vi "Set Translation.vi"(8 "error in (no error)":errorcluster, 9 "Default Lang":i32, 10 "Language":T1) -> (0 "error out":errorcluster)   [LabVIEW 2019, in "Language Selection.lvlib"]
doc: "Sets the translation of the VI controls according to the \"Language\" input index.\n- - -\nCopyright (c) 2026, Merecs Engineering GmbH"
uses:
  Language Selection.lvlib
  TypeDefs/Enum Language.ctl
  <vilib>/Utility/error.llb/Clear Errors.vi
  Set use unicode and default Lang.vi
  <vilib>/Utility/error.llb/Trim Whitespace.vi
  DVR Get Languages.vi
  Boolean Translate.vi
  Update Controls/Update MC Listbox vColumn headers.vi
  Update Controls/Update Listbox headers.vi
  Update Controls/Tool_Unicode Update Table Headers.vi
  Update Controls/update Graph.vi
  Update Controls/update 1D array.vi
  Update Controls/update tree column header.vi
  Update Controls/update 2D array.vi
  Update Controls/update listbox Items.vi
  Update Controls/update MultiColumn Listbox Items.vi
  Update Controls/Tool_Unicode Update Table Data.vi
  Update Controls/Update caption.vi
  Update Controls/update ring.vi
  <vilib>/addons/Tools/Unicode/Property Interpret As Unicode.vi
  <vilib>/addons/Tools/Unicode/Convert ASCII to UTF-16LE.vi
  <vilib>/addons/Tools/Unicode/_subVIs/Convert ASCII to UTF-16LE (1D).vi
  Update Controls/Update String value.vi
  Update Controls/Tool_Unicode Update Tab Control Pages.vi
  packages/error-generation/src/Error Generation/Add Argument.vi
panel:
  # "Connector Pane"
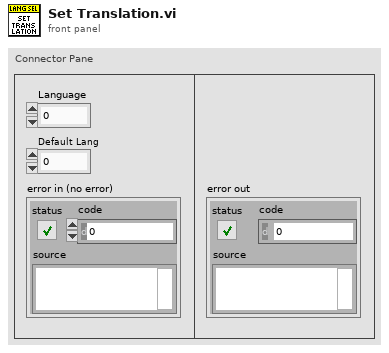
[diagram p1: front panel]
types:
  T1 = typedef "Language Selection.lvlib/Enum Language.ctl" = i32
  T2 = typedef "Language Selection.lvlib/Cluster LanguageClusterWithRefnum.ctl" = cluster{"Property":T3[], "Controls":set{refnum<vi>}}
  T3 = typedef "Language Selection.lvlib/Cluster PropertyTranslation.ctl" = cluster{"Type":T4, "Translation ANSI":string[], "Translation Unicode":string[]}
  T4 = typedef "Language Selection.lvlib/Enum Property Type.ctl" = enum16{"NA", "Caption", "String Value", "Boolean Text", "Ring Strings", "1D Array Elements", "2D Array Elements", "(MC)Listbox Header", "(MC)Listbox Items", "Tab Pages Names", "X & Y GraphChart", "Plot Names", "Table Headers", "Table Items", "TipStrip", "Combobox Strings", "Cursor Name", "Tree Col Headers"}
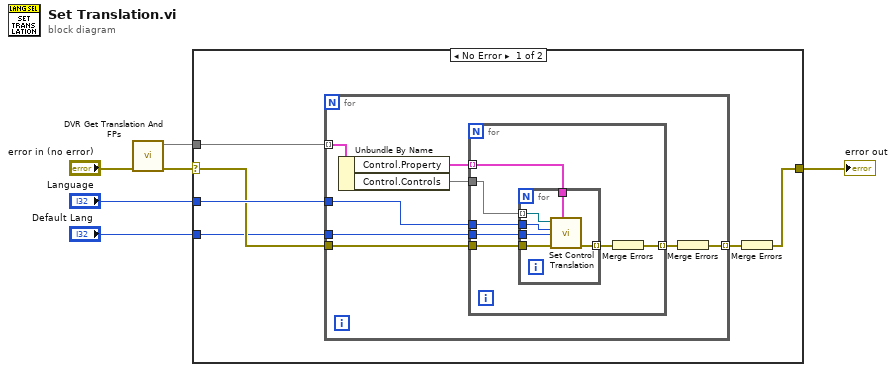
[diagram p0: block diagram]
diagram:
  n1 = call "DVR Get Translation And FPs.vi"("error in (no error)"="error in (no error)") -> ("error out"=w1:errorcluster, "FP Translation"=w3:map{string, T2})  [unwired: 8 in, 1 out]
  n2 = case shown="No Error" w1 {
    selector: w1 -> [w9 w34]
    tunnel: "Language" -> [w12 _]
    tunnel: [w11 w34] -> w5
    tunnel: w3 -> [w10 _]
    tunnel: "Default Lang" -> [w7 _]
    frame No Error {
      n3 = for {
        tunnel: w10 -> [w19] mode=indexing
        tunnel: w12 -> [w17]
        tunnel: w9 -> [w16]
        tunnel: [w14] -> w8 mode=indexing
        tunnel: w7 -> [w13]
        n4 = Unbundle By Name(w19) -> ("Control.Property"=w18:T3[], "Control.Controls"=w20:set{refnum<vi>})
        n5 = for {
          tunnel: w20 -> [w27]
          tunnel: w18 -> [w26] mode=indexing
          tunnel: w17 -> [w25]
          tunnel: w16 -> [w24]
          tunnel: [w22] -> w15 mode=indexing
          tunnel: w13 -> [w21]
          n6 = for {
            tunnel: w27 -> [w33] mode=indexing
            tunnel: w26 -> [w32]
            tunnel: w25 -> [w31]
            tunnel: w24 -> [w30]
            tunnel: [w29] -> w23 mode=indexing
            tunnel: w21 -> [w28]
            n7 = call "Set Control Translation.vi"("Obj."=w32, "error in (no error)"=w30, "Default Lang"=w28, "Language"=w31, "Control in"=w33) -> ("error out"=w29:errorcluster)  [unwired: 5 in, 1 out]
          }
          n8 = Merge Errors(w23) -> (w22:errorcluster)
        }
        n9 = Merge Errors(w15) -> (w14:errorcluster)
      }
      n10 = Merge Errors(w8) -> (w11:errorcluster)
    }
    frame Error {
    }
  }
  "error out" <- w5
